vi "Calculate Heater Values.vi"(0 "DAC HeatFlow AIV in":refnum<class "DAC HeatFlow AIV.lvclass">, 7 "dU Heater":dbl, 11 "error in":errorcluster) -> (4 "DAC HeatFlow AIV out":refnum<class "DAC HeatFlow AIV.lvclass">, 13 "dU Heater":dbl, 14 "P Heater":dbl, 15 "error out":errorcluster)   [LabVIEW 2019, in "DAC.lvlib" / "DAC HeatFlow AIV.lvclass"]
uses:
  DAC HeatFlow AIV.lvclass
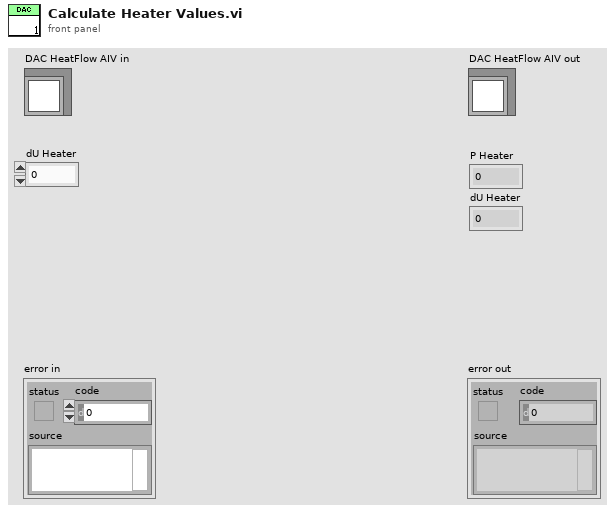
[diagram p1: front panel]
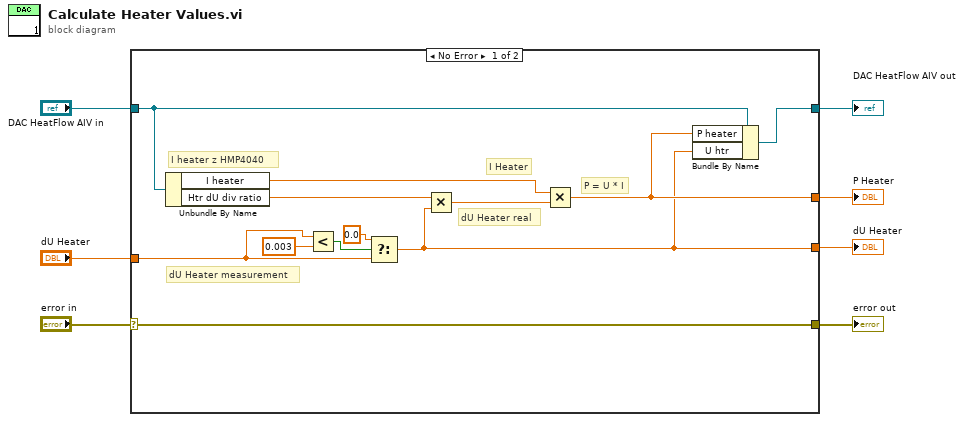
[diagram p0: block diagram]
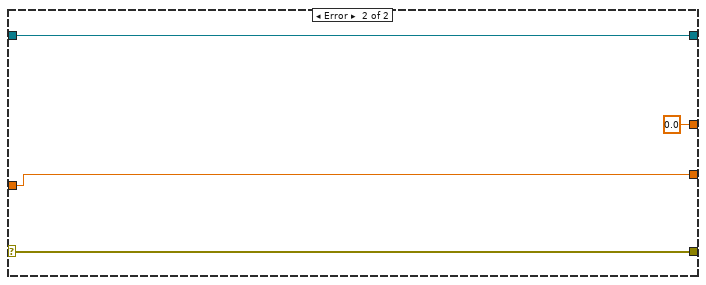
[diagram p2: hidden frame]
diagram:
  n1 = case shown="No Error" "error in" {
    selector: "error in" -> [w19 w23]
    tunnel: [w19 w23] -> w6
    tunnel: [w10 w22] -> w4
    tunnel: "DAC HeatFlow AIV in" -> [w18 w22]
    tunnel: "dU Heater" -> [w11 w21]
    tunnel: [w9 0.0] -> w2
    tunnel: [w8 w21] -> w1
    frame No Error {
      # "dU Heater measurement"
      # "I heater z HMP4040"
      # "I Heater"
      # "dU Heater real"
      # "P = U * I"
      n2 = Unbundle By Name(w18) -> ("I heater"=w12:dbl, "Htr dU div ratio"=w14:dbl)
      n3 = Less?(x=w11, y=0.003) -> (x < y?=w16:bool)
      n4 = Select(t=0.0, s=w16, f=w11) -> (s? t:f=w8:dbl)
      n5 = Multiply(x=w14, y=w8) -> (x*y=w13:dbl)
      n6 = Multiply(x=w12, y=w13) -> (x*y=w9:dbl)
      n7 = Bundle By Name(cluster=w18, "P heater"=w9, "U htr"=w8) -> (w10:refnum<class "DAC HeatFlow AIV.lvclass">)
    }
    frame Error {
    }
  }
  "error out" <- w6
  "DAC HeatFlow AIV out" <- w4
  "P Heater" <- w2
  "dU Heater" <- w1
